vi "Main Editor UI.vi"() -> ()   [LabVIEW 2014, in "SQLite editor node.lvclass"]
doc: "This is the main view for configuration the behavior of a module in the DCAF standard editor."
uses:
  SQLite editor node.lvclass
  <vilib>/NI/Configuration Framework/Node/NodeRef.ctl
  <vilib>/NI/Configuration Framework/Node/NISE_CEF_Node.lvclass
  <vilib>/NI/AMC/Message Queue.ctl
  <vilib>/NI/AMC/Message.ctl
  <vilib>/NI/Tools/Keyed Array/KeyedArray.ctl
  <vilib>/NI/Configuration Framework/Node/UserEventRef.ctl
  <vilib>/NI/Configuration Framework/Controls/EventCluster.ctl
  <vilib>/NI/DCAF UI Toolkit/Controls/Configure.ctl
  <vilib>/NI/DCAF UI Toolkit/Controls/Add.ctl
  <vilib>/NI/DCAF UI Toolkit/Controls/Remove.ctl
  <vilib>/NI/Configuration Framework/Node/StopEvent.ctl
  <vilib>/NI/Configuration Framework/Node/RefreshUIEvent.ctl
  <vilib>/NI/Configuration Framework/Node/CacheState.ctl
  <vilib>/NI/Configuration Framework/Node/NodeChangeEvent.ctl
  <vilib>/NI/Tag Bus/tag/Data Type.ctl
  Permissions Enum.ctl
  <vilib>/NI/DCAF/Tag Editor Core/Table API/Available Tag Menu/channel action event.ctl
  <vilib>/NI/DCAF/Tag Editor Core/Table API/Available Tag Menu/dialog output action.ctl
  <vilib>/NI/Tag Bus Module Framework/channel/TBM channel.lvclass
  <vilib>/NI/Tag Bus/tag/tag descriptor.lvclass
  <vilib>/NI/DCAF/Tag Editor Core/Table API/Table Manager/Call Back Ref Type Def.ctl
  <vilib>/NI/DCAF/Tag Editor Core/Configuration Editor/Classes/Engine Parent/Engine Parent Editor Node.lvclass
  <vilib>/NI/DCAF/Tag Editor Core/Configuration Editor/Classes/Module editor node/module editor node.lvclass
  <vilib>/NI/DCAF/Tag Editor Core/Table API/Table Manager/references.ctl
  <vilib>/Utility/miscctls.llb/LVPositionTypeDef.ctl
  <vilib>/NI/DCAF/Tag Editor Core/Table API/Listbox/Multi Column Listbox.lvclass
  <vilib>/NI/Configuration Framework/NISE_CEF_TreeControl.lvlib
  <vilib>/NI/Tools/Keyed Array/Tools_KeyedArray.lvlib
  <vilib>/NI/AMC/AMC.lvlib
  <vilib>/NI/DCAF/Tag Editor Core/Table API/Table Manager.lvlib
  <vilib>/NI/DCAF/Tag Editor Core/Table API/Table Manager/Table Manager.lvclass
  <vilib>/NI/DCAF UI Toolkit/Controls/DCAF UI Elements.lvlib
panel:
  in  "user event out":refnum<user-event>
  in  "Permissions":T1
  in  "data type":T2
  in  "node change":T3
  in  "cache state":T4
  in  "refresh UI":T5
  in  "stop event":T6
  in  "Tab Control":T7(tab)
  in  "Remove Button":T8
  in  "Add Button":T9
  in  "Table":i32(listbox)
  in  "settings":T10
  in  "Table Name":string
  in  "use default name?":bool=TRUE
  in  "Database File Name":string="sqlite.db"
  in  "Overwrite existing?":bool=TRUE
  in  "Log Directory":path
  in  "Log Directory":string
  in  "user event":T11
  in  "main queue":T12
  in  "node ref":T13
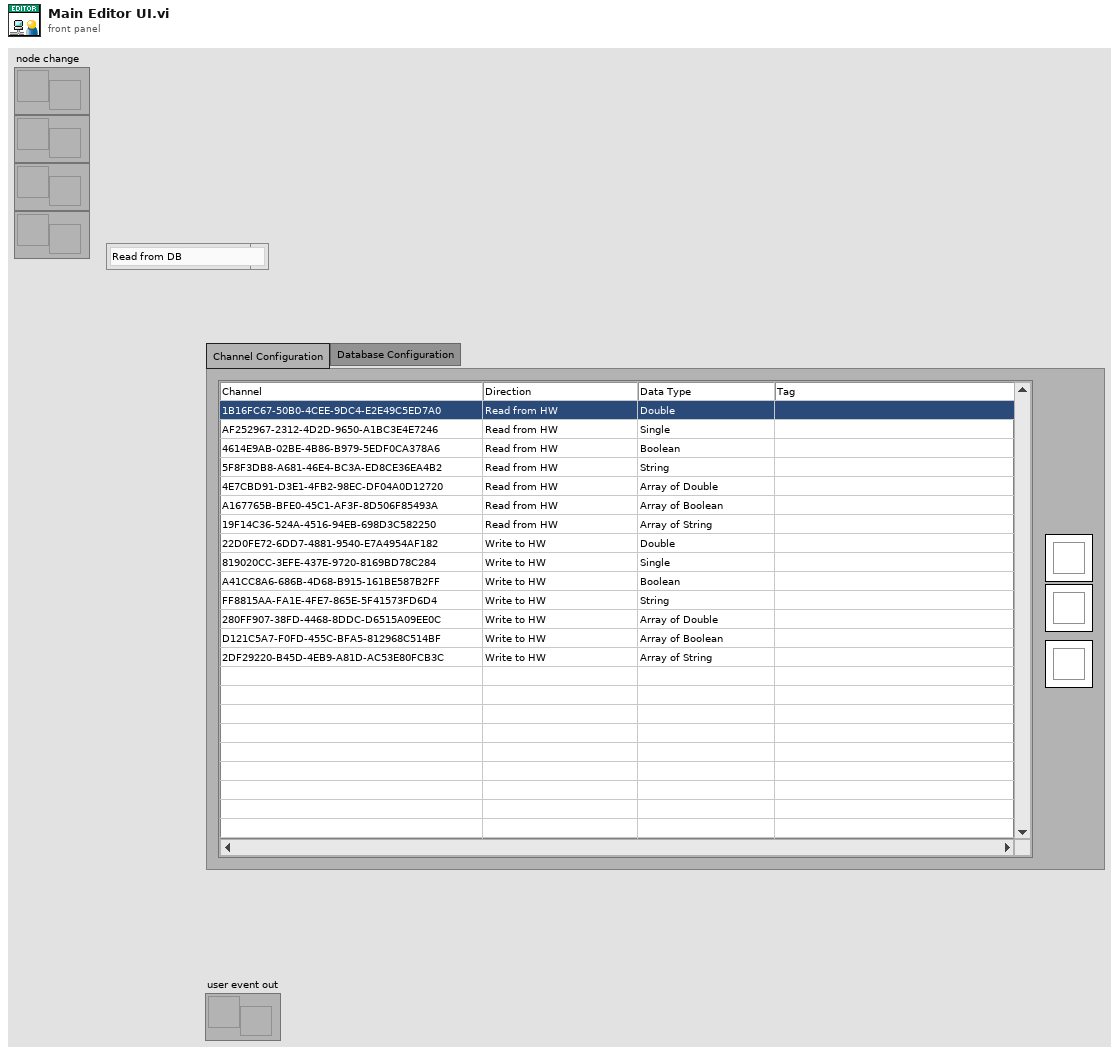
[diagram p1: front panel]
types:
  T1 = typedef "SQLite editor node.lvclass/Permissions Enum.ctl" = enum16{"Read from DB", "Write to DB"}
  T2 = typedef "tag bus.lvlib/tag descriptor.lvclass/Data Type.ctl" = enum16{"Double", "Single", "I64", "I32", "I16", "I8", "U64", "U32", "U16", "U8", "Boolean", "String", "Array of Double", "Array of Single", "Array of I64", "Array of I32", "Array of I16", "Array of I8", "Array of U64", "Array of U32", "Array of U16", "Array of U8", "Array of Boolean", "Array of String"}
  T3 = typedef "NISE_CEF_Node.lvclass/NodeChangeEvent.ctl" = refnum<user-event>
  T4 = typedef "NISE_CEF_Node.lvclass/CacheState.ctl" = refnum<user-event>
  T5 = typedef "NISE_CEF_Node.lvclass/RefreshUIEvent.ctl" = refnum<user-event>
  T6 = typedef "NISE_CEF_Node.lvclass/StopEvent.ctl" = refnum<user-event>
  T7 = enum32{"Channel Configuration", "Database Configuration"}
  T8 = typedef "DCAF UI Elements.lvlib/Remove.ctl" = bool
  T9 = typedef "DCAF UI Elements.lvlib/Add.ctl" = bool
  T10 = typedef "DCAF UI Elements.lvlib/Configure.ctl" = bool
  T11 = typedef "NISE_CEF_Node.lvclass/UserEventRef.ctl" = refnum<user-event>
  T12 = typedef "AMC.lvlib/Message Queue.ctl" = refnum<queue>
  T13 = typedef "NISE_CEF_Node.lvclass/NodeRef.ctl" = refnum<data-value>
  T14 = enum8{"Enabled", "Disabled", "Disabled and Grayed Out"}
  T15 = typedef "Table Manager.lvlib/Table Manager.lvclass/references.ctl" = cluster{"stop event":T6, "refresh UI":T5, "cache state":T4, "node change":T3, "user event out":refnum<user-event>, "main queue":T12, "user event":T11}
  T16 = typedef "LVPositionTypeDef.ctl" = cluster{"Left":i32, "Top":i32}
  T17 = typedef "Table Manager.lvlib/Table Manager.lvclass/object ref.ctl" = cluster{"engine":refnum<data-value>, "Node Ref":refnum<data-value>}
  T18 = typedef "Table Manager.lvlib/Column.lvclass/Column Descriptor.ctl" = cluster{"name":string, "caption":string, "Column Type":T19, "Params":string, "AutoSizeMode":i32, "FillWeight":sgl, "MinWidth":u32, "tooltip":string, "Enum Reference":refnum<vi>, "Channel suffix":string, "Read Only":bool, "Call Back VI":T20, "DT Dependency":i32, "name dependency":i32, "data type":T2, "Custom Column":refnum<class "Column.lvclass">}
  T19 = typedef "Table Manager.lvlib/Column.lvclass/Column Type.ctl" = enum16{"String", "Mapping", "Enum", "Custom"}
  T20 = typedef "Table Manager.lvlib/Table Manager.lvclass/Call Back Ref Type Def.ctl" = refnum<vi>
  T21 = typedef "TBM configuration.lvclass/Target Types.ctl" = enum16{"Windows", "Mac", "Linux", "Linux RT ARM", "VxWorks", "Pharlap", "Other", "Linux RT x64"}
  T22 = typedef "Table Manager.lvlib/Table Manager.lvclass/Table Events.ctl" = cluster{"Menu Selection":refnum<user-event>}
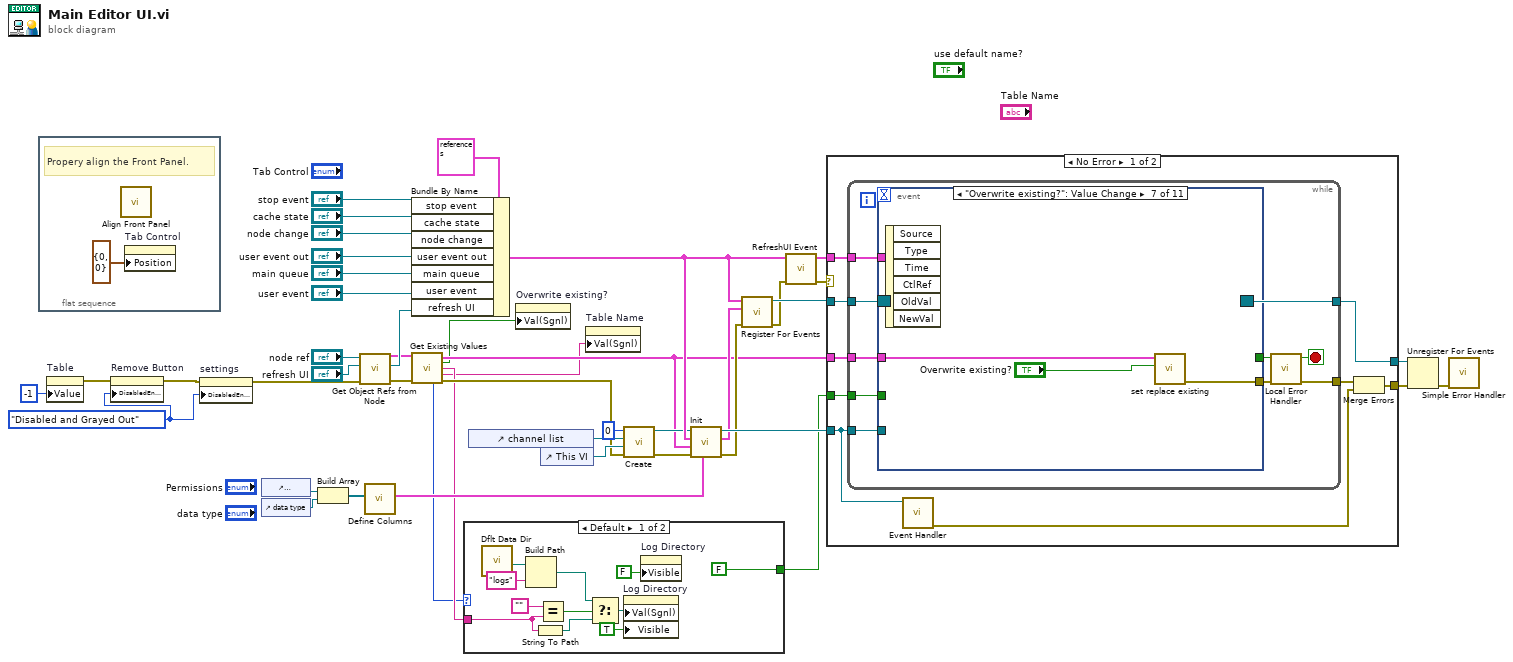
[diagram p0: block diagram]
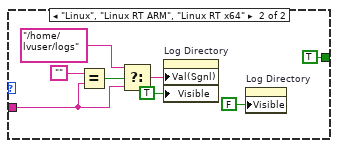
[diagram p2: hidden frame]
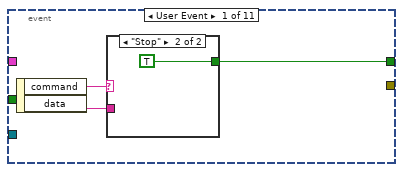
[diagram p3: hidden frame]
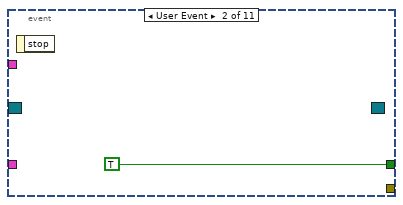
[diagram p5: hidden frame]
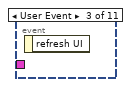
[diagram p6: hidden frame]
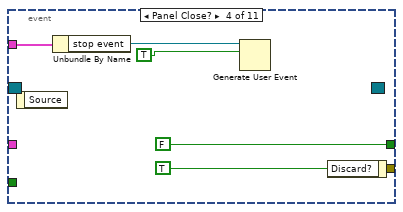
[diagram p7: hidden frame]
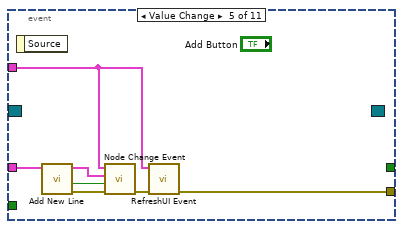
[diagram p8: hidden frame]
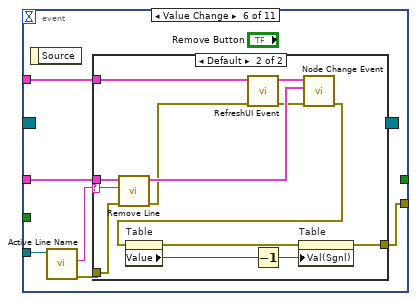
[diagram p9: hidden frame]
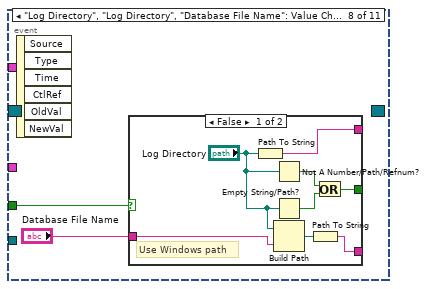
[diagram p11: hidden frame]
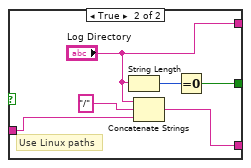
[diagram p12: hidden frame]
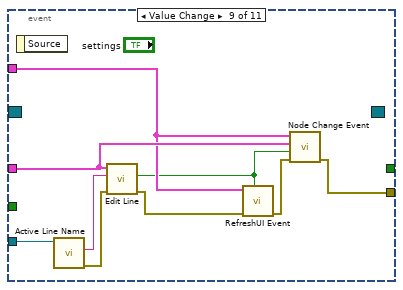
[diagram p13: hidden frame]
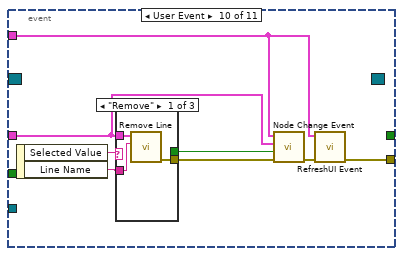
[diagram p14: hidden frame]
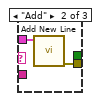
[diagram p15: hidden frame]
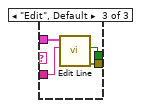
[diagram p16: hidden frame]
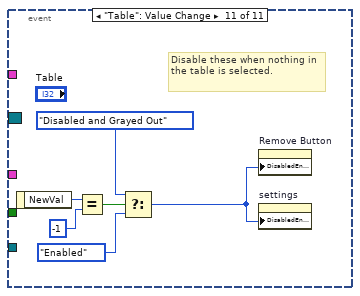
[diagram p17: hidden frame]
diagram:
  w11 = T14."Disabled and Grayed Out" ("Disabled")
  n1 = flat-sequence {
    frame #0 {
      # "Propery align the Front Panel."
      n2 = call <vilib>:"Align Front Panel.vi"() -> ()  [unwired: 10 in, 2 out]
      n3 = property on="Tab Control" class="TabCtl (strict)"("Position"=T16 {"Left"=0, "Top"=0}) -> ()  [unwired: 2 in, 2 out]
    }
  }
  n4 = property on="Table" class="MCListbox (strict)"("Value"=-1 ("Table")) -> (error out=w12:errorcluster)  [unwired: 2 in, 1 out]
  n5 = property on="Remove Button" class="Bool"(error in=w12, "DisabledEnum"=w11) -> (error out=w14:errorcluster)  [unwired: 1 in, 1 out]
  n6 = property on="settings" class="Bool"(error in=w14, "DisabledEnum"=w11) -> (error out=w10:errorcluster)  [unwired: 1 in, 1 out]
  n7 = control-ref of="Permissions"() -> (w30:refnum<vi>)
  n8 = control-ref of="data type"() -> (w29:refnum<vi>)
  n9 = Build Array(w30, w29) -> (w28:refnum<vi>[])
  n10 = call "Get Object Refs from Node.vi"("error in (no error)"=w10, "Refresh UI"="refresh UI", "Data Value Reference in"="node ref") -> ("error out"=w6:errorcluster, "Refresh UI out"=w15:T5, "References"=w8:T17)  [unwired: 6 in]
  n11 = call "Define Columns.vi"("Enum Array"=w28) -> ("Column Definition"=w33:T18[])  [unwired: 10 in]
  n12 = Bundle By Name(cluster=T15 {"stop event"=refnum, "refresh UI"=refnum, "cache state"=refnum, "node change"=refnum, "user event out"=refnum, "main queue"=refnum, "user event"=refnum} ("References"), "stop event"="stop event", "cache state"="cache state", "node change"="node change", "user event out"="user event out", "main queue"="main queue", "user event"="user event", "refresh UI"=w15) -> (w31:T15)
  n13 = call "Get Existing Values.vi"("References"=w8, "error in (no error)"=w6) -> ("References out"=w7:T17, "Replace existing"=w2:bool, "DB File Path"=w4:string, "Table Name"=w1:string, "Target Type"=w3:T21, "error out"=w5:errorcluster)  [unwired: 8 in]
  n14 = case shown="Default" w3 {
    tunnel: w4 -> [w48 w59]
    tunnel: [FALSE TRUE] -> w9
    frame Default {
      n15 = call <vilib>:"Dflt Data Dir.vi"() -> ("App:Default Data Directory"=w51:path)
      n16 = Build Path(base path=w51, name or relative path="logs") -> (appended path=w53:path)
      n17 = String To Path(string=w48) -> (path=w47:path)
      n18 = Equal?(x="", y=w48) -> (x = y?=w49:bool)
      n19 = Select(t=w53, s=w49, f=w47) -> (s? t:f=w46:path)
      n20 = property on="Log Directory" class="Path"("Val(Sgnl)"=w46, "Visible"=TRUE) -> ()  [unwired: 2 in, 2 out]
      n21 = property on="Log Directory" class="Str"("Visible"=FALSE) -> ()  [unwired: 2 in, 2 out]
    }
    frame "Linux", "Linux RT ARM", "Linux RT x64" {
      n22 = Equal?(x="", y=w59) -> (x = y?=w60:bool)
      n23 = Select(t="/home/lvuser/logs", s=w60, f=w59) -> (s? t:f=w58:string)
      n24 = property on="Log Directory" class="Str"("Val(Sgnl)"=w58, "Visible"=TRUE) -> ()  [unwired: 2 in, 2 out]
      n25 = property on="Log Directory" class="Path"("Visible"=FALSE) -> ()  [unwired: 2 in, 2 out]
    }
  }
  n26 = control-ref of="channel list"() -> (w21:refnum<vi>)
  n27 = property on="Overwrite existing?" class="Bool (strict)"("Val(Sgnl)"=w2) -> ()  [unwired: 2 in, 2 out]
  n28 = control-ref of="This VI"() -> (w19:refnum<vi>)
  n29 = property on="Table Name" class="Str"("Val(Sgnl)"=w1) -> ()  [unwired: 2 in, 2 out]
  n30 = call <vilib>:"Create.vi"("error in (no error)"=w5, "Top VI"=w19, "Listbox"=w21, "Index"=0) -> ("error out"=w17:errorcluster, "reference out"=w18:refnum<class "Multi Column Listbox.lvclass">)  [unwired: 6 in]
  n31 = call-dynamic "Init.vi"("Column Descriptors"=w33, "error in (no error)"=w17, "Node object refs"=w7, "Event References"=w31, "Multi Column Listbox in"=w18) -> ("error out"=w23:errorcluster, "Table Events"=w22:T22, "Multi Column Listbox out"=w27:refnum<class "Multi Column Listbox.lvclass">)  [unwired: 4 in]
  n32 = call "Register For Events.vi"("error in"=w23, "Table Events"=w22, "References"=w31) -> ("error out"=w25:errorcluster, "Event Registration Refnum"=w34:refnum<event-registration>)  [unwired: 7 in]
  n33 = call "RefreshUI Event.vi"("error in (no error)"=w25, "References in"=w31) -> ("error out"=w24:errorcluster, "References out"=w32:T15)  [unwired: 8 in]
  n34 = case shown="No Error" w24 {
    selector: w24 -> [_ w171]
    tunnel: w34 -> [w73 w170]
    tunnel: [w72 w170] -> w44
    tunnel: [w66 w171] -> w43
    tunnel: w32 -> [w71 _]
    tunnel: w7 -> [w70 _]
    tunnel: w27 -> [w69 _]
    tunnel: w9 -> [w65 _]
    frame No Error {
      n35 = while {
        tunnel: w73 -> [w83]
        tunnel: [w82] -> w72
        tunnel: [w79] -> w67
        tunnel: w71 -> [w77]
        tunnel: w70 -> [w76]
        tunnel: w69 -> [w75]
        tunnel: w65 -> [w74]
        stop <- w81 stop-if-true
        n36 = event shown="[6] \"Overwrite existing?\": Value Change" {
          selector: w83 -> [_ _ _ _ _ _ _ _ _ _ _]
          dyn-events: [_ _ _ _ _ _ _ _ _ _ _] -> w82
          timeout: _ -> [_ _ _ _ _ _ _ _ _ _ _]
          tunnel: [w86 TRUE _ FALSE _ _ _ _ _ _ _] -> w80
          tunnel: [_ _ _ _ w94 w101 w119 _ w146 w152 _] -> w78
          tunnel: w77 -> [_ _ _ w90 w98 w105 _ _ w141 w148 _]
          tunnel: w76 -> [_ _ _ _ w99 w104 w121 _ w144 w149 _]
          tunnel: w75 -> [_ _ _ _ _ w103 _ _ w145 _ _]
          tunnel: w74 -> [_ _ _ _ _ _ _ w122 _ _ _]
          event User Event {
            n37 = event-data() -> ("command"=w85:string, "data"=w84:string)  [unwired: 1 in]
            n38 = case shown="\"Stop\"" w85 {
              tunnel: [_ TRUE] -> w86
              tunnel: w84 -> [_ _]
              frame Default {
              }
              frame "Stop" {
              }
            }
          }
          event User Event {
            n39 = event-data() -> ()  [unwired: 1 in, 1 out]
          }
          event User Event {
            n40 = event-data() -> ()  [unwired: 1 in, 1 out]
          }
          event Panel Close? {
            n41 = event-data() -> ()  [unwired: 1 in, 1 out]
            n42 = Unbundle By Name(w90) -> ("stop event"=w89:T6)
            n43 = Generate User Event(user event=w89, event data cluster=TRUE ("event data")) -> ()  [unwired: 2 in, 2 out]
            n44 = event-data("Discard?"=TRUE) -> ()  [unwired: 1 in, 1 out]
          }
          event Value Change {
            n45 = event-data() -> ()  [unwired: 1 in, 1 out]
            n46 = call "Add New Line.vi"("objects"=w99) -> ("error out"=w97:errorcluster, "success"=w95:bool)  [unwired: 8 in, 1 out]
            n47 = call "Node Change Event.vi"("error in (no error)"=w97, "Send (T)"=w95, "objects"=w99, "References in"=w98) -> ("error out"=w96:errorcluster)  [unwired: 7 in]
            n48 = call "RefreshUI Event.vi"("error in (no error)"=w96, "References in"=w98) -> ("error out"=w94:errorcluster)  [unwired: 8 in, 1 out]
          }
          event Value Change {
            n49 = event-data() -> ()  [unwired: 1 in, 1 out]
            n50 = call-dynamic "Active Line Name.vi"("Multi Column Listbox in"=w103) -> ("error out"=w102:errorcluster, "Active Line Name"=w100:string)  [unwired: 8 in, 1 out]
            n51 = case shown="Default" w100 {
              selector: w100 -> [_ w107]
              tunnel: w105 -> [_ w118]
              tunnel: w104 -> [_ w117]
              tunnel: w102 -> [w106 w113]
              tunnel: [w106 w109] -> w101
              frame "" {
                # "Blank line name = tried to \nremove a line that does not exist"
              }
              frame Default {
                n52 = call "Remove Line.vi"("error in"=w113, "Active Line Name"=w107, "Objects"=w117) -> ("error out"=w114:errorcluster)  [unwired: 8 in]
                n53 = call "RefreshUI Event.vi"("error in (no error)"=w114, "References in"=w118) -> ("error out"=w116:errorcluster, "References out"=w115:T15)  [unwired: 8 in]
                n54 = call "Node Change Event.vi"("error in (no error)"=w116, "objects"=w117, "References in"=w115) -> ("error out"=w110:errorcluster)  [unwired: 8 in]
                n55 = property on="Table" class="MCListbox (strict)"(error in=w110) -> (error out=w108:errorcluster, "Value"=w111:i32)  [unwired: 1 in, 1 out]
                n56 = Decrement(x=w111) -> (x-1=w112:i32)
                n57 = property on="Table" class="MCListbox (strict)"(error in=w108, "Val(Sgnl)"=w112) -> (error out=w109:errorcluster)  [unwired: 1 in, 1 out]
              }
            }
          }
          event "Overwrite existing?": Value Change {
            n58 = event-data() -> ()  [unwired: 1 in, 6 out]
            n59 = call "set replace existing.vi"("Replace existing"="Overwrite existing?", "References"=w121) -> ("error out"=w119:errorcluster)  [unwired: 8 in, 1 out]
          }
          event "Log Directory", "Log Directory", "Database File Name": Value Change {
            n60 = event-data() -> ()  [unwired: 1 in, 6 out]
            n61 = case shown="False" w122 {
              tunnel: [w129 w136] -> _
              tunnel: [w128 "Log Directory"] -> _
              tunnel: "Database File Name" -> [w126 w134]
              tunnel: [w124 w132] -> _
              frame False {
                # "Use Windows path"
                n62 = Path To String(path="Log Directory") -> (string=w128:string)
                n63 = Not A Number/Path/Refnum?(number/path/refnum="Log Directory") -> (NaN/Path/Refnum?=w130:bool)
                n64 = Empty String/Path?(string/path="Log Directory") -> (empty?=w131:bool)
                n65 = Build Path(base path="Log Directory", name or relative path=w126) -> (appended path=w125:path)
                n66 = Path To String(path=w125) -> (string=w124:string)
                n67 = Or(x=w130, y=w131) -> (x .or. y?=w129:bool)
              }
              frame True {
                # "Use Linux paths"
                n68 = String Length(string="Log Directory") -> (length=w137:i32)
                n69 = Concatenate Strings("Log Directory", "/" ("string"), w134) -> (w132:string)
                n70 = Equal To 0?(x=w137) -> (x = 0?=w136:bool)
              }
            }
          }
          event Value Change {
            n71 = event-data() -> ()  [unwired: 1 in, 1 out]
            n72 = call-dynamic "Active Line Name.vi"("Multi Column Listbox in"=w145) -> ("error out"=w142:errorcluster, "Active Line Name"=w143:string)  [unwired: 8 in, 1 out]
            n73 = call "Edit Line.vi"("error in"=w142, "Line Name"=w143, "References"=w144) -> ("error out"=w139:errorcluster, "change?"=w140:bool)  [unwired: 7 in]
            n74 = call "RefreshUI Event.vi"("Refresh (T)"=w140, "error in (no error)"=w139, "References in"=w141) -> ("error out"=w138:errorcluster)  [unwired: 7 in, 1 out]
            n75 = call "Node Change Event.vi"("error in (no error)"=w138, "Send (T)"=w140, "objects"=w144, "References in"=w141) -> ("error out"=w146:errorcluster)  [unwired: 7 in]
          }
          event User Event {
            n76 = event-data() -> ("Selected Value"=w154:string, "Line Name"=w151:string)  [unwired: 1 in]
            n77 = case shown="\"Remove\"" w154 {
              tunnel: w151 -> [w157 _ w163]
              tunnel: w149 -> [w156 w159 w162]
              tunnel: [w155 w158 w161] -> w150
              tunnel: [_ _ w160] -> w147
              frame "Remove" {
                n78 = call "Remove Line.vi"("Active Line Name"=w157, "Objects"=w156) -> ("error out"=w155:errorcluster)  [unwired: 9 in]
              }
              frame "Add" {
                n79 = call "Add New Line.vi"("objects"=w159) -> ("error out"=w158:errorcluster)  [unwired: 8 in, 2 out]
              }
              frame "Edit", Default {
                n80 = call "Edit Line.vi"("Line Name"=w163, "References"=w162) -> ("error out"=w161:errorcluster, "change?"=w160:bool)  [unwired: 8 in]
              }
            }
            n81 = call "Node Change Event.vi"("error in (no error)"=w150, "Send (T)"=w147, "objects"=w149, "References in"=w148) -> ("error out"=w153:errorcluster)  [unwired: 7 in]
            n82 = call "RefreshUI Event.vi"("error in (no error)"=w153, "References in"=w148) -> ("error out"=w152:errorcluster)  [unwired: 8 in, 1 out]
          }
          event "Table": Value Change {
            # "Disable these when nothing in the table is selected."
            n83 = event-data() -> ("NewVal"=w169:i32)  [unwired: 1 in]
            n84 = Equal?(x=w169, y=-1) -> (x = y?=w167:bool)
            n85 = Select(t=T14."Disabled and Grayed Out" ("Disabled"), s=w167, f=T14."Enabled") -> (s? t:f=w165:T14)
            n86 = property on="Remove Button" class="Bool"("DisabledEnum"=w165) -> ()  [unwired: 2 in, 2 out]
            n87 = property on="settings" class="Bool"("DisabledEnum"=w165) -> ()  [unwired: 2 in, 2 out]
          }
        }
        n88 = call "Local Error Handler.vi"("error in"=w78, "Stop in"=w80) -> ("error out"=w79:errorcluster, "Stop out"=w81:bool)  [unwired: 8 in]
      }
      n89 = call-dynamic "Event Handler.vi"("Listbox in"=w69) -> ("error out"=w68:errorcluster)  [unwired: 9 in, 1 out]
      n90 = Merge Errors(w67, w68) -> (w66:errorcluster)
    }
    frame Error {
    }
  }
  n91 = Unregister For Events(event registration refnum=w44, error in=w43) -> (error out=w42:errorcluster)
  n92 = call <vilib>:"Simple Error Handler.vi"("error in (no error)"=w42) -> ()  [unwired: 4 in, 5 out]
